vi "Acquisition - Apply Calibration.vi"(8 "error in (no error)":errorcluster) -> (0 "error out":errorcluster)   [LabVIEW 2026, in "Unit Tests.lvlib"]
uses:
  Unit Tests.lvlib
  Libraries/CML Shared/Calibration Values--cluster.ctl
  <vilib>/addons/_JKI Toolkits/Caraya/classes/Assert/Assert True.vi
  Libraries/Acquisition/Acquisition.lvlib
  Libraries/CML Shared/CML Shared.lvlib
  <vilib>/addons/_JKI Toolkits/Caraya/classes/Test/Test.lvclass
  <vilib>/addons/_JKI Toolkits/Caraya/classes/Assert/Assert.lvclass
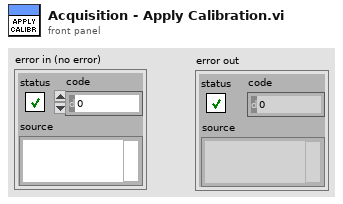
[diagram p1: front panel]
types:
  T1 = typedef "CML Shared.lvlib/Calibration Values--cluster.ctl" = cluster{"Slope":dbl, "Offset":dbl}
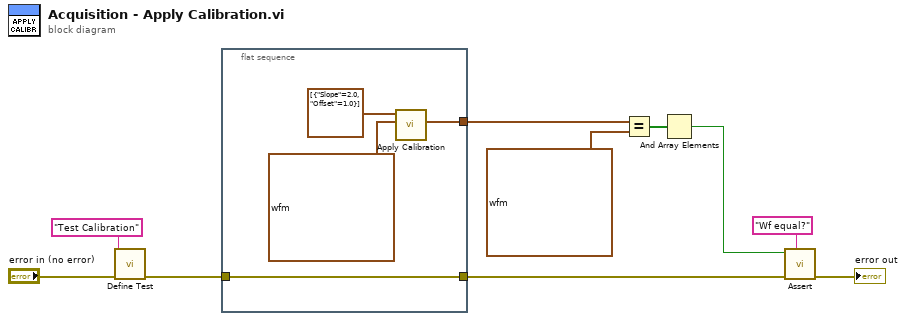
[diagram p0: block diagram]
diagram:
  n1 = call <vilib>:"Define Test.vi"("error in (no error)"="error in (no error)", "Label (VI Title)"="Test Calibration") -> ("error out"=w10:errorcluster)  [unwired: 8 in, 1 out]
  n2 = flat-sequence {
    tunnel: w10 -> [w12]
    tunnel: [w12] -> w9
    tunnel: [w11] -> w8
    frame #0 {
      n3 = call "Apply Calibration.vi"("Graph Data"=waveform(dbl)[] [{"t0"=timestamp(0 s since 1904-01-01), "dt"=1.0, "Y"=[10.0]}], "Calibration Array"=T1[] [{"Slope"=2.0, "Offset"=1.0}]) -> ("Calibrated Data"=w11:waveform(dbl)[])  [unwired: 9 in]
    }
  }
  n4 = Equal?(x=w8, y=waveform(dbl)[] [{"t0"=timestamp(0 s since 1904-01-01), "dt"=1.0, "Y"=[21.0]}] ("Graph Data")) -> (x = y?=w6:bool[])
  n5 = And Array Elements(Boolean array=w6) -> (logical AND=w5:bool)
  n6 = call-poly <vilib>:"Assert.vi"("Label"="Wf equal?", "error in (no error)"=w9, "True?"=w5) -> ("error out"=→"error out":errorcluster)  [unwired: 7 in, 1 out]
